vi "Load Stage Limits.vi"() -> (4 "Notifier Names":string[](array[string]), 8 "Stage Limits":T1[](array[typedef]), 15 "Loaded":bool)   [LabVIEW 2016]
uses:
  Stages Limits Type Defs/Stage Limits.ctl
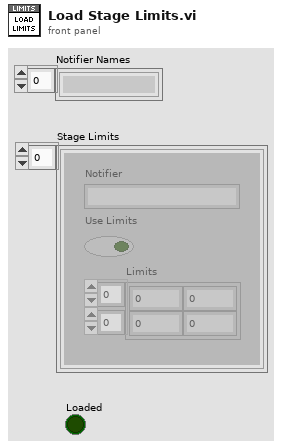
[diagram p1: front panel]
types:
  T1 = typedef "Stage Limits.ctl" = cluster{"Notifier":string, "Use Limits":bool, "Limits":dbl[][]}
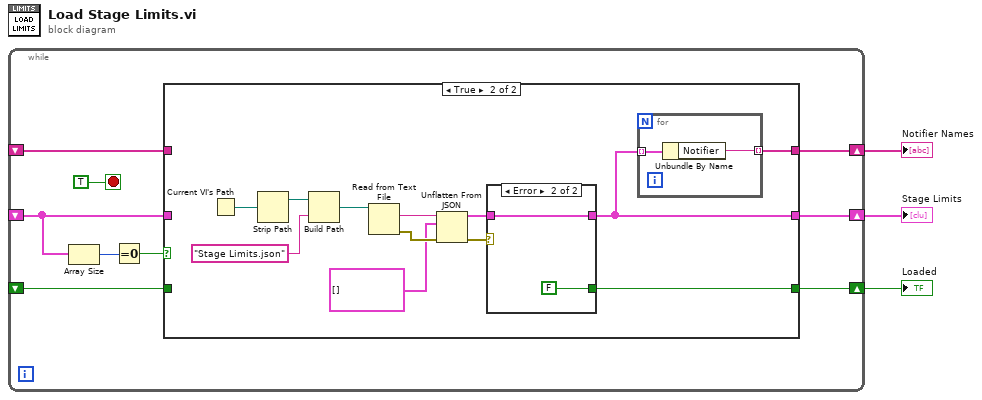
[diagram p0: block diagram]
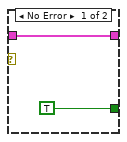
[diagram p3: hidden frame]
diagram:
  n1 = while {
    shift-right: [w11] -> w3
    shift-left: _ -> [w8]
    shift-right: [w7] -> w2
    shift-left: _ -> [w6]
    shift-right: [w5] -> w1
    shift-left: _ -> [w4]
    stop <- TRUE stop-if-true
    n2 = Array Size(array=w8) -> (size(s)=w10:i32)
    n3 = Equal To 0?(x=w10) -> (x = 0?=w9:bool)
    n4 = case shown="True" w9 {
      tunnel: [w15 w18] -> w11
      tunnel: w8 -> [w15 _]
      tunnel: [w14 w19] -> w7
      tunnel: w6 -> [w14 _]
      tunnel: [w13 w17] -> w5
      tunnel: w4 -> [w13 _]
      frame False {
      }
      frame True {
        n5 = Current VI's Path() -> (path=w16:path)
        n6 = Strip Path(path=w16) -> (stripped path=w27:path)  [unwired: 1 out]
        n7 = Build Path(base path=w27, name or relative path="Stage Limits.json") -> (appended path=w21:path)
        n8 = Read from Text File(file (use dialog)=w21) -> (text=w25:string, error out=w24:errorcluster)  [unwired: 3 in, 2 out]
        n9 = Unflatten From JSON(JSON string=w25, type and defaults=T1[] [], error in (no error)=w24) -> (value=w22:T1[], error out=w23:errorcluster)  [unwired: 4 in]
        n10 = case shown="Error" w23 {
          tunnel: w22 -> [w31 w33]
          tunnel: [w31 w33] -> w18
          tunnel: [TRUE FALSE] -> w19
          frame No Error {
          }
          frame Error {
          }
        }
        n11 = for {
          tunnel: w18 -> [w29] mode=indexing
          tunnel: [w28] -> w17 mode=indexing
          n12 = Unbundle By Name(w29) -> ("Notifier"=w28:string)
        }
      }
    }
  }
  "Stage Limits" <- w3
  "Loaded" <- w2
  "Notifier Names" <- w1
